vi "InstalPlotStile (SubVI).vi"(10 "StileIn":T1(array[cluster])=[{"Plot.Bar Plot Style"=0, "Plot.DigitalLineStyle"=1, "Plot.Line Style"=0, "Plot.Line Width"=2, "Plot.Plot Color"=5863167, "Plot.Plot Name"="Plot 0", "Plot.Point Style"=0}, {"Plot.Bar Plot Style"=0, "Plot.DigitalLineStyle"=1, "Plot.Line Style"=0, "Plot.Line Width"=2, "Plot.Plot Color"=13257796, "Plot.Plot Name"="Plot 1", "Plot.Point Style"=0}, {"Plot.Bar Plot Style"=0, "Plot.DigitalLineStyle"=1, "Plot.Line Style"=0, "Plot.Line Width"=2, "Plot.Plot Color"=6601816, "Plot.Plot Name"="Plot 2", "Plot.Point Style"=0}, {"Plot.Bar Plot Style"=0, "Plot.DigitalLineStyle"=1, "Plot.Line Style"=0, "Plot.Line Width"=2, "Plot.Plot Color"=15441725, "Plot.Plot Name"="Plot 3", "Plot.Point Style"=0}, {"Plot.Bar Plot Style"=0, "Plot.DigitalLineStyle"=1, "Plot.Line Style"=0, "Plot.Line Width"=2, "Plot.Plot Color"=8742822, "Plot.Plot Name"="Plot 4", "Plot.Point Style"=0}, {"Plot.Bar Plot Style"=0, "Plot.DigitalLineStyle"=1, "Plot.Line Style"=0, "Plot.Line Width"=3, "Plot.Plot Color"=10051840, "Plot.Plot Name"="Plot 5", "Plot.Point Style"=0}, {"Plot.Bar Plot Style"=0, "Plot.DigitalLineStyle"=1, "Plot.Line Style"=0, "Plot.Line Width"=3, "Plot.Plot Color"=3121844, "Plot.Plot Name"="Plot 6", "Plot.Point Style"=0}, {"Plot.Bar Plot Style"=0, "Plot.DigitalLineStyle"=1, "Plot.Line Style"=0, "Plot.Line Width"=3, "Plot.Plot Color"=13592771, "Plot.Plot Name"="Plot 7", "Plot.Point Style"=0}, {"Plot.Bar Plot Style"=0, "Plot.DigitalLineStyle"=1, "Plot.Line Style"=0, "Plot.Line Width"=3, "Plot.Plot Color"=931427, "Plot.Plot Name"="Plot 8", "Plot.Point Style"=0}, {"Plot.Bar Plot Style"=0, "Plot.DigitalLineStyle"=1, "Plot.Line Style"=0, "Plot.Line Width"=3, "Plot.Plot Color"=9014678, "Plot.Plot Name"="Plot 9", "Plot.Point Style"=0}, {"Plot.Bar Plot Style"=0, "Plot.DigitalLineStyle"=1, "Plot.Line Style"=0, "Plot.Line Width"=0, "Plot.Plot Color"=14483242, "Plot.Plot Name"="Plot 10", "Plot.Point Style"=0}, {"Plot.Bar Plot Style"=0, "Plot.DigitalLineStyle"=1, "Plot.Line Style"=0, "Plot.Line Width"=1, "Plot.Plot Color"=9538739, "Plot.Plot Name"="Plot 11", "Plot.Point Style"=0}, {"Plot.Bar Plot Style"=0, "Plot.DigitalLineStyle"=1, "Plot.Line Style"=0, "Plot.Line Width"=0, "Plot.Plot Color"=982784, "Plot.Plot Name"="Plot 12", "Plot.Point Style"=0}, {"Plot.Bar Plot Style"=0, "Plot.DigitalLineStyle"=1, "Plot.Line Style"=0, "Plot.Line Width"=0, "Plot.Plot Color"=4375295, "Plot.Plot Name"="Plot 13", "Plot.Point Style"=0}, {"Plot.Bar Plot Style"=0, "Plot.DigitalLineStyle"=1, "Plot.Line Style"=0, "Plot.Line Width"=0, "Plot.Plot Color"=13827953, "Plot.Plot Name"="Plot 14", "Plot.Point Style"=0}, {"Plot.Bar Plot Style"=0, "Plot.DigitalLineStyle"=1, "Plot.Line Style"=0, "Plot.Line Width"=0, "Plot.Plot Color"=13457919, "Plot.Plot Name"="Plot 15", "Plot.Point Style"=0}, {"Plot.Bar Plot Style"=0, "Plot.DigitalLineStyle"=1, "Plot.Line Style"=0, "Plot.Line Width"=0, "Plot.Plot Color"=16757522, "Plot.Plot Name"="Plot 16", "Plot.Point Style"=0}, {"Plot.Bar Plot Style"=0, "Plot.DigitalLineStyle"=1, "Plot.Line Style"=0, "Plot.Line Width"=0, "Plot.Plot Color"=4343295, "Plot.Plot Name"="Plot 17", "Plot.Point Style"=0}, {"Plot.Bar Plot Style"=0, "Plot.DigitalLineStyle"=1, "Plot.Line Style"=0, "Plot.Line Width"=0, "Plot.Plot Color"=16728758, "Plot.Plot Name"="Plot 18", "Plot.Point Style"=0}, {"Plot.Bar Plot Style"=0, "Plot.DigitalLineStyle"=1, "Plot.Line Style"=0, "Plot.Line Width"=0, "Plot.Plot Color"=5898228, "Plot.Plot Name"="Plot 19", "Plot.Point Style"=0}], 11 "XYGraph in":refnum<vi>) -> ()   [LabVIEW 2017]
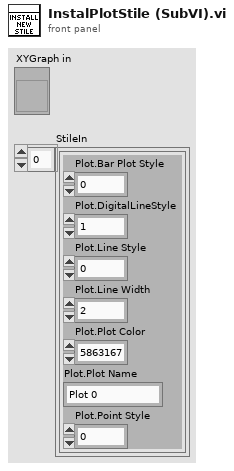
[diagram p1: front panel]
types:
  T1 = cluster{"Plot.Bar Plot Style":u8, "Plot.DigitalLineStyle":u8, "Plot.Line Style":u8, "Plot.Line Width":u8, "Plot.Plot Color":u32, "Plot.Plot Name":string, "Plot.Point Style":u8}[]
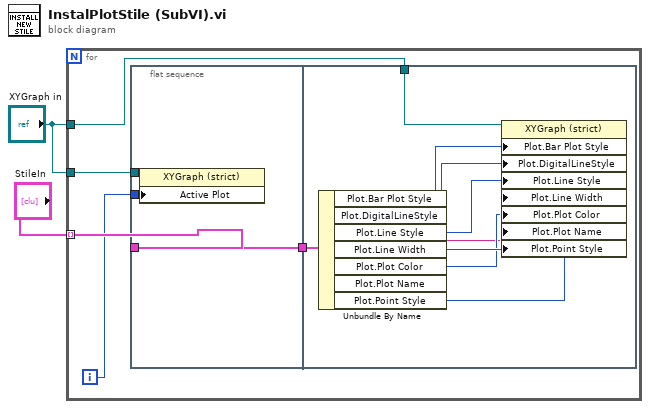
[diagram p0: block diagram]
diagram:
  n1 = for {
    tunnel: "StileIn" -> [w7] mode=indexing
    tunnel: "XYGraph in" -> [w4]
    tunnel: "XYGraph in" -> [w3]
    i -> [w5]
    n2 = flat-sequence {
      tunnel: w7 -> [w10]
      tunnel: [w10] -> w6
      tunnel: w5 -> [w9]
      tunnel: w3 -> [w8]
      tunnel: w6 -> [w12]
      tunnel: w4 -> [w11]
      frame #0 {
        n3 = property on="Property Node" class="XYGraph (strict)"(reference=w8, "Active Plot"=w9) -> ()  [unwired: 1 in, 2 out]
      }
      frame #1 {
        n4 = Unbundle By Name(w12) -> ("Plot.Bar Plot Style"=w19:u8, "Plot.DigitalLineStyle"=w18:u8, "Plot.Line Style"=w17:u8, "Plot.Line Width"=w16:u8, "Plot.Plot Color"=w15:u32, "Plot.Plot Name"=w14:string, "Plot.Point Style"=w13:u8)
        n5 = property on="Property Node" class="XYGraph (strict)"(reference=w11, "Plot.Bar Plot Style"=w19, "Plot.DigitalLineStyle"=w18, "Plot.Line Style"=w17, "Plot.Line Width"=w16, "Plot.Plot Color"=w15, "Plot.Plot Name"=w14, "Plot.Point Style"=w13) -> ()  [unwired: 1 in, 2 out]
      }
    }
  }
